vi "Sprite_Blit.vi"(0 "Picture":u8[][](array[numeric]), 5 "Sprites":cluster{"Pix":u8[][], "Mask":u8[][]}[](array[cluster]), 7 "Index":i32, 9 "Position":cluster{"X":i32, "Y":i32}, 11 "error in":errorcluster) -> (4 "Picture out":u8[][](array[numeric]), 15 "error out":errorcluster)   [LabVIEW 2020, in "GH_Render.lvlib"]
doc: "Copies Sprites[Index] with its mask (bytes 255/0, mixed bitwise) into the screen raster (720 rows x 1280*3 bytes RGB) so that its top left corner is at Position (X, Y); the part outside the screen is cut off (Y = -2000 hides a sprite)."
uses:
  GH_Render.lvlib
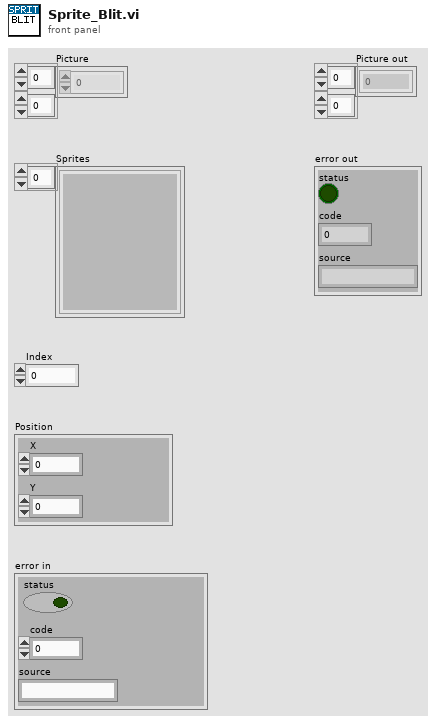
[diagram p1: front panel]
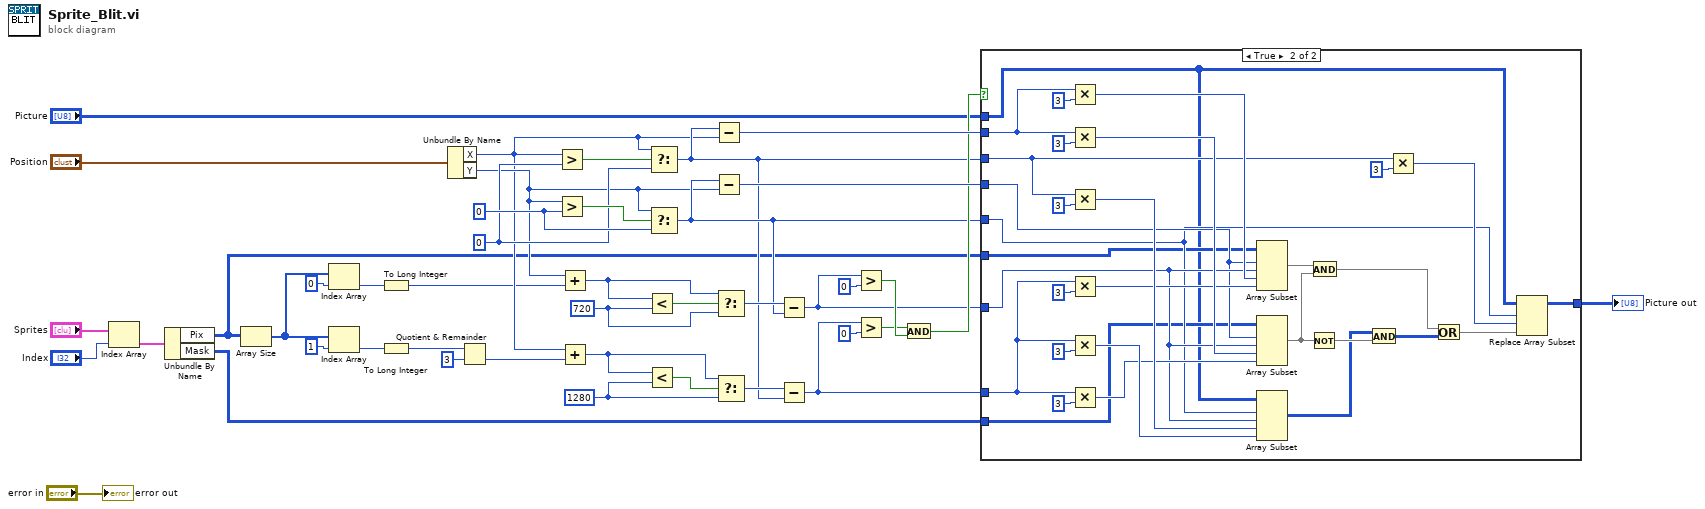
[diagram p0: block diagram]
diagram:
  w31 = 720
  w27 = 1280
  w23 = 0
  w20 = 0
  n1 = Index Array(array="Sprites", index="Index") -> (element=w6:cluster{"Pix":u8[][], "Mask":u8[][]})
  n2 = Unbundle By Name(w6) -> ("Pix"=w7:u8[][], "Mask"=w8:u8[][])
  n3 = Array Size(array=w7) -> (size(s)=w9:i32[])
  n4 = Index Array(array=w9, index=0) -> (element=w11:i32)
  n5 = Index Array(array=w9, index=1) -> (element=w14:i32)
  n6 = To Long Integer(number=w11) -> (32bit integer=w12:i32)
  n7 = To Long Integer(number=w14) -> (32bit integer=w15:i32)
  n8 = Unbundle By Name("Position") -> ("X"=w18:i32, "Y"=w19:i32)
  n9 = Quotient & Remainder(x=w15, y=3) -> (floor(x/y)=w17:i32)  [unwired: 1 out]
  n10 = Greater?(x=w18, y=w20) -> (0:w21:bool)
  n11 = Greater?(x=w19, y=w23) -> (0:w24:bool)
  n12 = Add(x=w19, y=w12) -> (x+y=w30:i32)
  n13 = Add(x=w18, y=w17) -> (x+y=w26:i32)
  n14 = Less?(x=w30, y=w31) -> (x < y?=w32:bool)
  n15 = Less?(x=w26, y=w27) -> (x < y?=w28:bool)
  n16 = Select(t=w18, s=w21, f=w20) -> (s? t:f=w22:i32)
  n17 = Select(t=w19, s=w24, f=w23) -> (s? t:f=w25:i32)
  n18 = Subtract(x=w22, y=w18) -> (x-y=w41:i32)
  n19 = Subtract(x=w25, y=w19) -> (x-y=w42:i32)
  n20 = Select(t=w30, s=w32, f=w31) -> (s? t:f=w33:i32)
  n21 = Select(t=w26, s=w28, f=w27) -> (s? t:f=w29:i32)
  n22 = Subtract(x=w33, y=w25) -> (x-y=w35:i32)
  n23 = Subtract(x=w29, y=w22) -> (x-y=w34:i32)
  n24 = Greater?(x=w35, y=0) -> (0:w39:bool)
  n25 = Greater?(x=w34, y=0) -> (0:w37:bool)
  n26 = And(x=w37, y=w39) -> (x .and. y?=w40:bool)
  n27 = case shown="True" w40 {
    tunnel: "Picture" -> [w44 w45]
    tunnel: w7 -> [_ w46]
    tunnel: w8 -> [_ w47]
    tunnel: w22 -> [_ w48]
    tunnel: w25 -> [_ w49]
    tunnel: w41 -> [_ w50]
    tunnel: w42 -> [_ w51]
    tunnel: w35 -> [_ w53]
    tunnel: w34 -> [_ w52]
    tunnel: [w44 w75] -> w43
    frame False {
    }
    frame True {
      n28 = Multiply(x=w50, y=3) -> (x*y=w55:i32)
      n29 = Multiply(x=w50, y=3) -> (x*y=w60:i32)
      n30 = Multiply(x=w48, y=3) -> (x*y=w65:i32)
      n31 = Multiply(x=w52, y=3) -> (x*y=w57:i32)
      n32 = Multiply(x=w52, y=3) -> (x*y=w67:i32)
      n33 = Multiply(x=w52, y=3) -> (x*y=w62:i32)
      n34 = Array Subset(array=w46, index (row)=w51, length (row)=w53, index (col)=w55, length (col)=w57) -> (w58:u8[][])
      n35 = Array Subset(array=w47, index (row)=w51, length (row)=w53, index (col)=w60, length (col)=w62) -> (w63:u8[][])
      n36 = Array Subset(array=w45, index (row)=w49, length (row)=w53, index (col)=w65, length (col)=w67) -> (w68:u8[][])
      n37 = Not(x=w63) -> (.not. x?=w70:u8[][])
      n38 = And(x=w58, y=w63) -> (x .and. y?=w69:u8[][])
      n39 = And(x=w68, y=w70) -> (x .and. y?=w71:u8[][])
      n40 = Multiply(x=w48, y=3) -> (x*y=w74:i32)
      n41 = Or(x=w69, y=w71) -> (x .or. y?=w72:u8[][])
      n42 = Replace Array Subset(array=w45, new element=w72, index (row)=w49, index (col)=w74) -> (w75:u8[][])
    }
  }
  "Picture out" <- w43
  "error out" <- "error in"
